vi "写控件文本.vi"(6 "数组":string[][](array[string]), 9 "字号":u32, 10 "选择列":i32, 11 "引用":refnum<vi>) -> ()   [LabVIEW 2025]
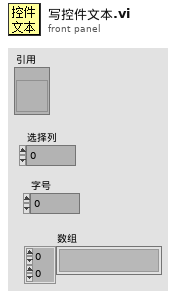
[diagram p1: front panel]
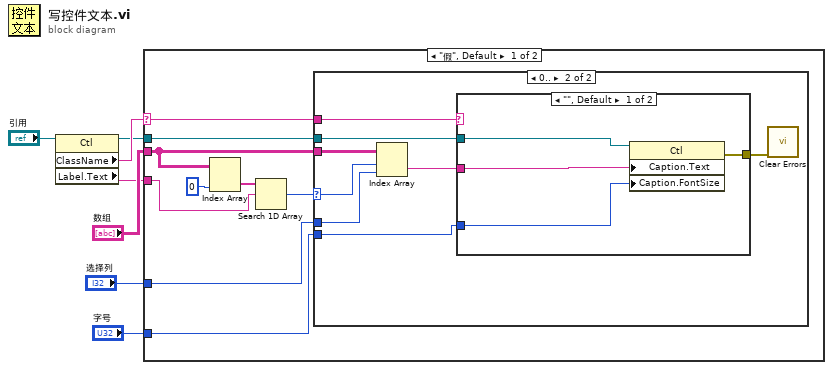
[diagram p0: block diagram]
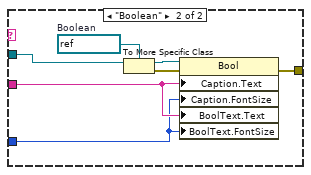
[diagram p3: hidden frame]
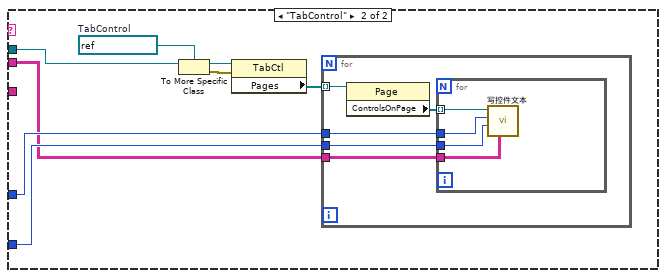
[diagram p4: hidden frame]
diagram:
  n1 = property class="Ctl"(reference="引用") -> (reference out=w3:refnum<vi>, "ClassName"=w4:string, "Label.Text"=w2:string)  [unwired: 1 in, 1 out]
  n2 = case shown="\"假\", Default" w4 {
    selector: w4 -> [w16 _]
    tunnel: w3 -> [w15 w42]
    tunnel: "数组" -> [w10 w36]
    tunnel: w2 -> [w12 _]
    tunnel: "选择列" -> [w9 w38]
    tunnel: "字号" -> [w8 w37]
    frame "假", Default {
      n3 = Index Array(array=w10, index (col)=0 ("禁用的索引 (列)")) -> (element=w13:string[])  [unwired: 1 in]
      n4 = Search 1D Array(1D array=w13, element=w12) -> (index of element=w11:i32)  [unwired: 1 in]
      n5 = case shown="0.." w11 {
        selector: w11 -> [_ w21]
        tunnel: w16 -> [_ w24]
        tunnel: w15 -> [_ w23]
        tunnel: w10 -> [_ w22]
        tunnel: w9 -> [_ w20]
        tunnel: w8 -> [_ w18]
        frame -1, Default {
        }
        frame 0.. {
          n6 = Index Array(array=w22, index (row)=w21, index (col)=w20) -> (element=w19:string)
          n7 = case shown="\"\", Default" w24 {
            tunnel: w23 -> [w28 w35]
            tunnel: w19 -> [w27 w31]
            tunnel: w18 -> [w26 w30]
            tunnel: [w25 w29] -> w17
            frame "", Default {
              n8 = property class="Ctl"(reference=w28, "Caption.Text"=w27, "Caption.FontSize"=w26) -> (error out=w25:errorcluster)  [unwired: 1 in, 1 out]
            }
            frame "Boolean" {
              w32 = refnum<vi> refnum  # Boolean
              n9 = To More Specific Class(target class=w32, reference=w35) -> (specific class reference=w34:refnum<vi>, error out=w33:errorcluster)  [unwired: 1 in]
              n10 = property class="Bool"(reference=w34, error in=w33, "Caption.Text"=w31, "Caption.FontSize"=w30, "BoolText.Text"=w31, "BoolText.FontSize"=w30) -> (error out=w29:errorcluster)  [unwired: 1 out]
            }
          }
          n11 = call <vilib>:"Clear Errors.vi"("error in (no error)"=w17) -> ()  [unwired: 5 in, 2 out]
        }
      }
    }
    frame "TabControl" {
      w43 = refnum<vi> refnum  # TabControl
      n12 = To More Specific Class(target class=w43, reference=w42) -> (specific class reference=w41:refnum<vi>, error out=w40:errorcluster)  [unwired: 1 in]
      n13 = property class="TabCtl"(reference=w41, error in=w40) -> ("Pages"=w39:refnum<vi>[])  [unwired: 2 out]
      n14 = for {
        tunnel: w39 -> [w48] mode=indexing
        tunnel: w38 -> [w46]
        tunnel: w37 -> [w45]
        tunnel: w36 -> [w44]
        n15 = property class="Page"(reference=w48) -> ("ControlsOnPage"=w47:refnum<vi>[])  [unwired: 1 in, 2 out]
        n16 = for {
          tunnel: w47 -> [w52] mode=indexing
          tunnel: w46 -> [w51]
          tunnel: w45 -> [w50]
          tunnel: w44 -> [w49]
          n17 = call "写控件文本.vi"("数组"=w49, "字号"=w50, "选择列"=w51, "引用"=w52) -> ()  [unwired: 8 in]
        }
      }
    }
  }
